vi "Compute Destination Endpoints.vi"(8 "error in":errorcluster, 9 "endpoints":string[](array[string]), 10 "source endpoint":string, 11 "instrument handle in":refnum<k15>) -> (0 "error out":errorcluster, 1 "existing destinations":string[](array[string]), 2 "available destinations":string[](array[string]), 3 "instrument handle out":refnum<k15>)   [LabVIEW 2020, in "NI-SWITCH Scripting.lvlib"]
uses:
  NI-SWITCH Scripting.lvlib
  <instrlib>/niSwitch/niSwitch.llb/niSwitch Path Capability.ctl
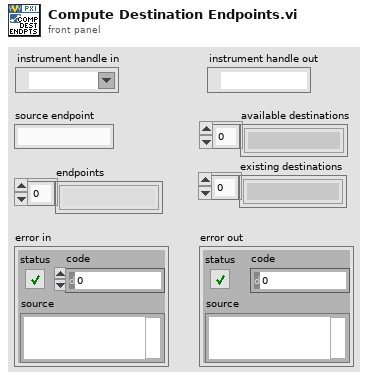
[diagram p1: front panel]
types:
  T1 = typedef "niSwitch Path Capability.ctl" = i32
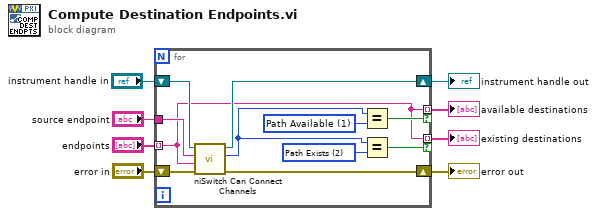
[diagram p0: block diagram]
diagram:
  n1 = for {
    tunnel: "endpoints" -> [w10] mode=indexing
    shift-right: [w18] -> w6
    shift-left: "error in" -> [w19]
    shift-right: [w16] -> w2
    shift-left: "instrument handle in" -> [w17]
    tunnel: "source endpoint" -> [w15]
    tunnel: [w10] -> w8 mode=indexing if=w14
    tunnel: [w10] -> w1 mode=indexing if=w9
    w12 = T1 2 items=["Path Available"=1, "Path Exists"=2, "Path Unsupported"=3, "Resource in Use"=4, "Source Conflict"=5, "Channel Not Available"=6] ("path capability")
    w13 = T1 1 items=["Path Available"=1, "Path Exists"=2, "Path Unsupported"=3, "Resource in Use"=4, "Source Conflict"=5, "Channel Not Available"=6] ("path capability")
    n2 = call <instrlib>:"niSwitch Can Connect Channels.vi"("error in (no error)"=w19, "channel 2"=w10, "channel 1"=w15, "instrument handle"=w17) -> ("error out"=w18:errorcluster, "path capability"=w11:T1, "instrument handle out"=w16:refnum<k15>)  [unwired: 5 in]
    n3 = Equal?(x=w11, y=w13) -> (x = y?=w14:bool)
    n4 = Equal?(x=w11, y=w12) -> (x = y?=w9:bool)
  }
  "available destinations" <- w8
  "error out" <- w6
  "instrument handle out" <- w2
  "existing destinations" <- w1
